vi "Attach Role Policy.vi"(8 "error in (no error)":errorcluster, 9 "Policy ARN":string, 10 "Role Name":string, 11 "IAM Session in":refnum<class "IAM Session.lvclass">) -> (0 "error out":errorcluster, 3 "IAM Session out":refnum<class "IAM Session.lvclass">)   [LabVIEW 2015, in "NI_AWS_IAM.lvlib" / "IAM Session.lvclass"]
uses:
  IAM Session.lvclass
  Core/HTTP Request/Request Options.ctl
  Core/HTTP Request/Name Value Pair.ctl
  Core/HTTP Request/Region handling.ctl
  Core/HTTP Request/URL formatting.ctl
  Core/HTTP Request/HTTP Request.lvclass
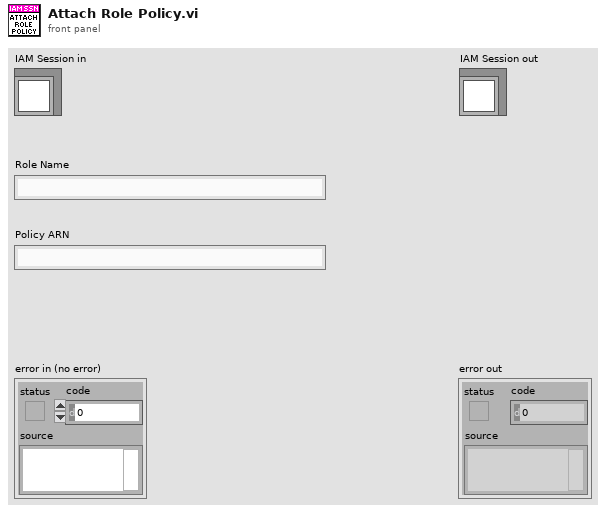
[diagram p1: front panel]
types:
  T1 = typedef "NI_AWS_Core.lvlib/HTTP Request.lvclass/Name Value Pair.ctl" = cluster{"name":string, "value":string}
  T2 = typedef "NI_AWS_Core.lvlib/HTTP Request.lvclass/Request Options.ctl" = cluster{"request headers":T1[], "request parameters":T1[], "request body":string, "region handling":T3, "URL formatting":T4}
  T3 = typedef "NI_AWS_Core.lvlib/HTTP Request.lvclass/Region handling.ctl" = enum16{"use region everywhere", "use region (authentication only)", "use region (URL only)", "ignore region everwhere"}
  T4 = typedef "NI_AWS_Core.lvlib/HTTP Request.lvclass/URL formatting.ctl" = enum16{"region-", "region."}
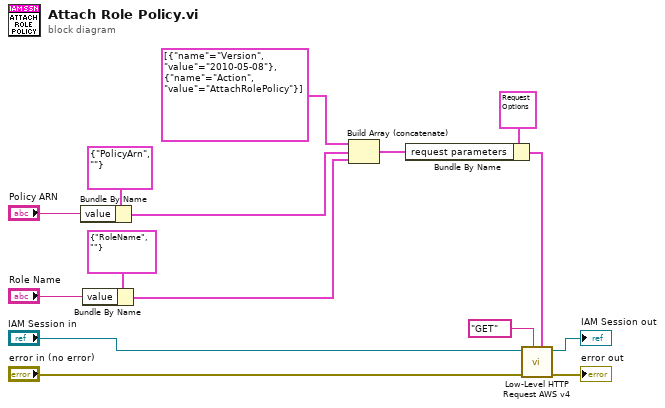
[diagram p0: block diagram]
diagram:
  n1 = Bundle By Name(cluster=T1 {"name"="PolicyArn", "value"=""} ("Name Value Pair"), "value"="Policy ARN") -> (w2:T1)
  n2 = Bundle By Name(cluster=T1 {"name"="RoleName", "value"=""} ("Name Value Pair"), "value"="Role Name") -> (w1:T1)
  n3 = Build Array (concatenate)(T1[] [{"name"="Version", "value"="2010-05-08"}, {"name"="Action", "value"="AttachRolePolicy"}], w2, w1) -> (w7:T1[])
  n4 = Bundle By Name(cluster=T2 {"request headers"=[], "request parameters"=[], "request body"="", "region handling"=enum."use region everywhere", "URL formatting"=enum."region."} ("Request Options"), "request parameters"=w7) -> (w9:T2)
  n5 = call "Low-Level HTTP Request AWS v4.vi"("Request Options"=w9, "HTTP-Verb"="GET", "error in (no error)"="error in (no error)", "AWS Core in"="IAM Session in") -> ("error out"=→"error out":errorcluster, "AWS Core out"=→"IAM Session out":refnum<class "IAM Session.lvclass">)  [unwired: 4 in, 2 out]
